vi "GDSAPI_Example_AddDesignPattern.vi"() -> ()   [LabVIEW 2020]
uses:
  GDSAPI_SubVIs/GDSAPI_ClassProviderType.ctl
  ClassProviders/Common/String/GDSString_MethodDescriptionType.ctl
  ClassProviders/Common/CommonVIs/CommonVIs_AttributeType.ctl
  ClassProviders/Common/CommonVIs/CommonVIs_AttributeDataType.ctl
  ClassProviders/Common/String/GDSString_AccessScopeModifierType.ctl
  ClassProviders/Common/String/GDSString_ModifierType.ctl
  ClassProviders/Common/CommonVIs/CommonVIs_PropertyType.ctl
  GDSAPI_CreateClassType.ctl
  GDSAPI_SubVIs/GDSAPI_ClassTemplateType.ctl
  GDSAPI_CreateInterfaceType.ctl
  ClassProviders/Provider_BaseClassInterface/ClassWriter_class/InterfaceMethodsToCreate.ctl
  ClassProviders/Provider_BaseClassInterface/ClassWriter_class/ClassWriter.lvclass
panel:
  out "error out":errorcluster
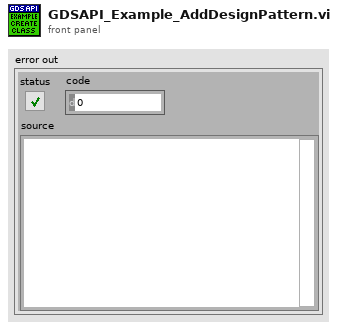
[diagram p1: front panel]
types:
  T1 = typedef "GDSString_MethodDescriptionType.ctl" = cluster{"ReturnType":T2, "MethodName":string, "AccessScope":T4, "Modifiers":T5[], "MethodDocumentation":string, "MethodContent":string, "MethodArguments":T2[], "GetProperty":T6, "SetProperty":T6}
  T2 = typedef "CommonVIs_AttributeType.ctl" = cluster{"Name":string, "DataType":T3, "ArrayDim":i32, "CtrlPath":path, "DataTypeString":string, "AccessScope":T4, "InitialData":variant}
  T3 = typedef "CommonVIs_AttributeDataType.ctl" = enum16{"UINT8", "INT8", "UINT16", "INT16", "UINT32", "INT32", "UINT64", "INT64", "SGL", "DBL", "EXT", "CSG", "CDB", "CXT", "TimeStamp", "STRING", "PATH", "BOOL", "ENUM", "RefNum", "VIRefNum", "LabVIEW Class", "Cluster", "Variant", "TypeDef", "Waveform", "LabVIEW Object", "Other", "void", "Set", "Map"}
  T4 = typedef "GDSString_AccessScopeModifierType.ctl" = enum16{"public", "private", "protected", "internal"}
  T5 = typedef "GDSString_ModifierType.ctl" = enum16{"abstract", "static", "final", "synchronized", "strictfp", "async", "const", "event", "extern", "new", "native ", "override", "partial", "readonly", "sealed", "unsafe", "virtual", "volatile"}
  T6 = typedef "CommonVIs_PropertyType.ctl" = cluster{"Active":bool, "AccessScope":T4, "Code":string}
  T7 = typedef "GDSAPI_ClassProviderType.ctl" = enum16{"LabVIEW Native(By value)", "GOOP-3(By reference)", "GOOP-4(By reference)"}
  T8 = typedef "GDSAPI_CreateInterfaceType.ctl" = cluster{"NewInterfaceFolder":path, "InterfaceName":string, "InterfaceDescription":string, "ParentInterfacesFilePath":path[], "FolderSuffix":string, "MethodsToCreate":T9[]}
  T9 = typedef "ClassWriter.lvclass/InterfaceMethodsToCreate.ctl" = cluster{"Name":string, "Description":string, "MethodsArgumentsIn":T2[], "MethodsArgumentsOut":T2[], "DecendantsMustOverride":bool}
  T10 = typedef "GDSAPI_CreateClassType.ctl" = cluster{"ClassProvider":T7, "NewClassFolder":path, "ParentLvClassFilePath":path, "ClassName":string, "ClassDescription":string, "ClassTemplate":T11, "ParentInterfacesFilePath":path[]}
  T11 = typedef "GDSAPI_ClassTemplateType.ctl" = enum16{"Standard", "Singleton"}
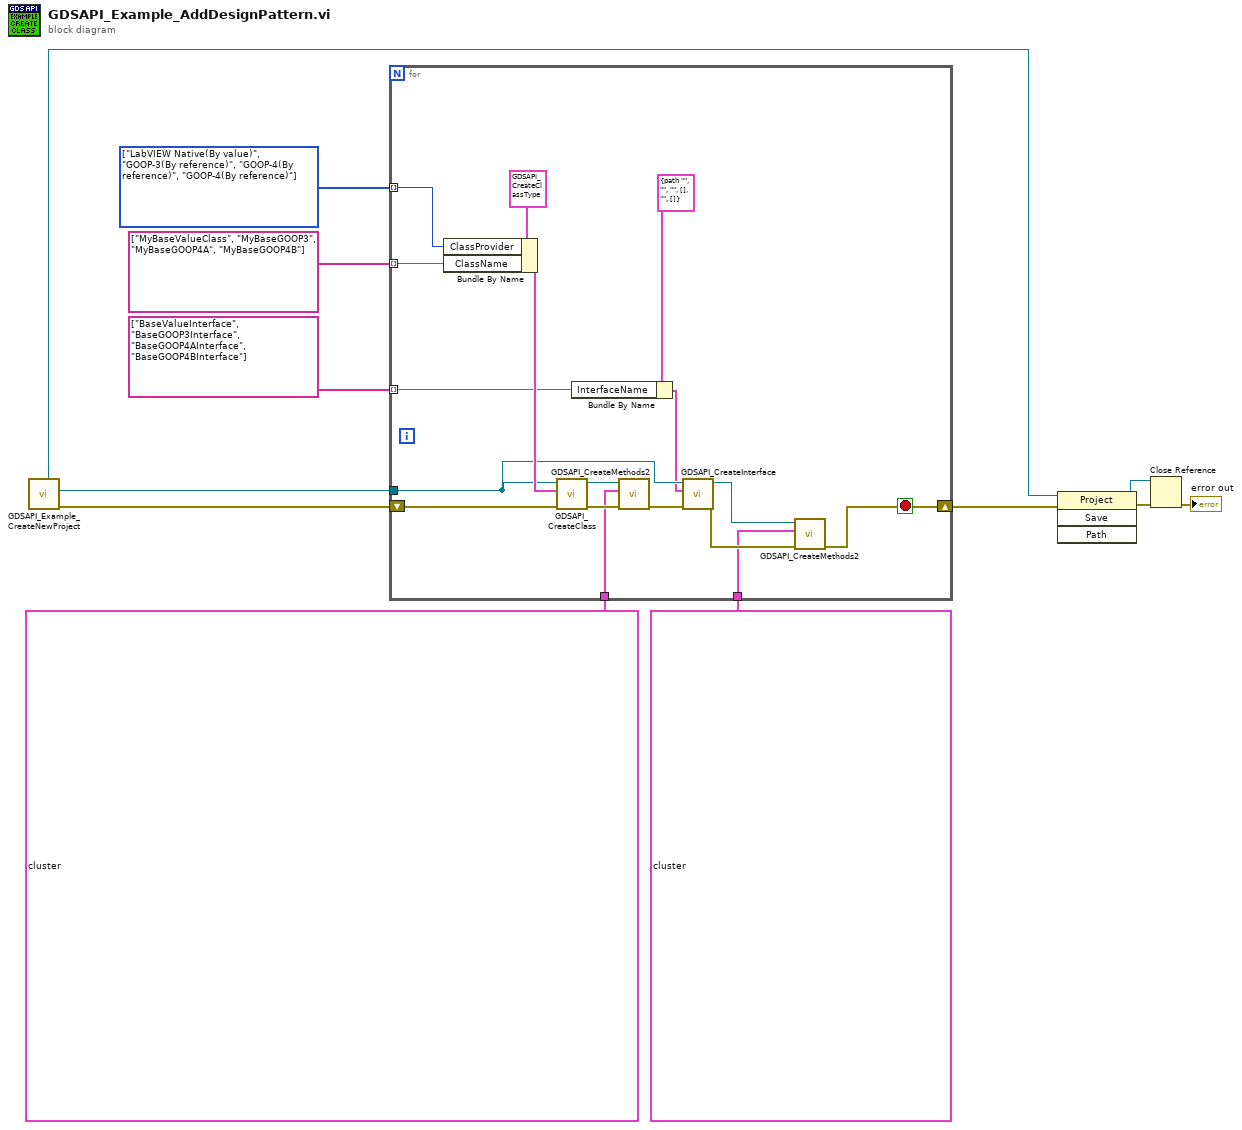
[diagram p0: block diagram]
diagram:
  w7 = T7[] [enum."LabVIEW Native(By value)", enum."GOOP-3(By reference)", enum."GOOP-4(By reference)", enum."GOOP-4(By reference)"] items=["LabVIEW Native(By value)", "GOOP-3(By reference)", "GOOP-4(By reference)"]
  n1 = call "GDSAPI_Example_CreateNewProject.vi"() -> ("error out"=w12:errorcluster, "ProjectItem out"=w11:refnum<vi>, "ProjectRefOut"=w6:refnum<vi>)  [unwired: 8 in, 1 out]
  n2 = for {
    tunnel: w11 -> [w24]
    tunnel: string[] ["MyBaseValueClass", "MyBaseGOOP3", "MyBaseGOOP4A", "MyBaseGOOP4B"] -> [w29] mode=indexing
    tunnel: w7 -> [w28] mode=indexing
    shift-right: [w15] -> w4
    shift-left: w12 -> [w27]
    tunnel: string[] ["BaseValueInterface", "BaseGOOP3Interface", "BaseGOOP4AInterface", "BaseGOOP4BInterface"] -> [w13] mode=indexing
    tunnel: T1[] [{"ReturnType"={"Name"="Message", "DataType"=enum."STRING", "ArrayDim"=0, "CtrlPath"=path "", "DataTypeString"="", "AccessScope"=enum."public", "InitialData"=variant}, "MethodName"="GetMessage", "AccessScope"=enum."public", "Modifiers"=[], "MethodDocumentation"="Doc Doc", "MethodContent"="static void Main()\n{\n    foreach (int number in SomeNumbers())\n    {\n        Console.Write(number.ToString() + \" \");\n    }\n    // Output: 3 5 8\n    Console.ReadKey();\n}", "MethodArguments"=[{"Name"="Get", "DataType"=enum."BOOL", "ArrayDim"=0, "CtrlPath"=path "", "DataTypeString"="", "AccessScope"=enum."public", "InitialData"=variant}], "GetProperty"={"Active"=FALSE, "AccessScope"=enum."public", "Code"=""}, "SetProperty"={"Active"=FALSE, "AccessScope"=enum."public", "Code"=""}}, {"ReturnType"={"Name"="Message", "DataType"=enum."STRING", "ArrayDim"=0, "CtrlPath"=path "", "DataTypeString"="", "AccessScope"=enum."public", "InitialData"=variant}, "MethodName"="GetMessage", "AccessScope"=enum."public", "Modifiers"=[], "MethodDocumentation"="Doc Doc", "MethodContent"="static void Main()\n{\n    foreach (int number in SomeNumbers())\n    {\n        Console.Write(number.ToString() + \" \");\n    }\n    // Output: 3 5 8\n    Console.ReadKey();\n}", "MethodArguments"=[{"Name"="Get", "DataType"=enum."BOOL", "ArrayDim"=0, "CtrlPath"=path "", "DataTypeString"="", "AccessScope"=enum."public", "InitialData"=variant}], "GetProperty"={"Active"=FALSE, "AccessScope"=enum."public", "Code"=""}, "SetProperty"={"Active"=FALSE, "AccessScope"=enum."public", "Code"=""}}] ("Methods") -> [w22]
    tunnel: T1[] [{"ReturnType"={"Name"="Number", "DataType"=enum."DBL", "ArrayDim"=0, "CtrlPath"=path "", "DataTypeString"="", "AccessScope"=enum."public", "InitialData"=variant}, "MethodName"="Do", "AccessScope"=enum."public", "Modifiers"=[], "MethodDocumentation"="My Doc", "MethodContent"=" public int Inventory\n  {\n    get\n    {\n       return _int;\n    }\n    set\n    {\n       // Just to make sure that if there is an increase in inventory then only we are notifying \n          the observers.\n          if (value > _int)\n             Notify();\n          _int = value;\n    }\n  }", "MethodArguments"=[{"Name"="A", "DataType"=enum."UINT8", "ArrayDim"=0, "CtrlPath"=path "", "DataTypeString"="", "AccessScope"=enum."public", "InitialData"=variant}, {"Name"="B", "DataType"=enum."UINT64", "ArrayDim"=1, "CtrlPath"=path "", "DataTypeString"="", "AccessScope"=enum."public", "InitialData"=variant}, {"Name"="C", "DataType"=enum."PATH", "ArrayDim"=0, "CtrlPath"=path "", "DataTypeString"="", "AccessScope"=enum."public", "InitialData"=variant}], "GetProperty"={"Active"=FALSE, "AccessScope"=enum."public", "Code"=""}, "SetProperty"={"Active"=FALSE, "AccessScope"=enum."public", "Code"=""}}] ("Methods") -> [w20]
    stop <- w15 stop-if-true
    n3 = Bundle By Name(cluster=T10 {"ClassProvider"=enum."LabVIEW Native(By value)", "NewClassFolder"=path "", "ParentLvClassFilePath"=path "", "ClassName"="", "ClassDescription"="", "ClassTemplate"=enum."Standard", "ParentInterfacesFilePath"=[]} ("CreateClassType"), "ClassProvider"=w28, "ClassName"=w29) -> (w25:T10)
    n4 = call "GDSAPI_CreateClass.vi"("error in (no error)"=w27, "CreateClassType"=w25, "ProjectItemToCreateClassUnder"=w24) -> ("error out"=w26:errorcluster, "LvClassFileOut"=w18:path)  [unwired: 6 in, 1 out]
    n5 = Bundle By Name(cluster=T8 {"NewInterfaceFolder"=path "", "InterfaceName"="", "InterfaceDescription"="", "ParentInterfacesFilePath"=[], "FolderSuffix"="", "MethodsToCreate"=[]} ("CreateInterfaceType"), "InterfaceName"=w13) -> (w14:T8)
    n6 = call "GDSAPI_CreateMethods2.vi"("error in (no error)"=w26, "Methods"=w22, "ClassPath(*.lvclass)"=w18) -> ("error out"=w23:errorcluster)  [unwired: 7 in, 1 out]
    n7 = call "GDSAPI_CreateInterface.vi"("error in (no error)"=w23, "CreateInterfaceType"=w14, "ProjectItemToCreateClassUnder"=w24) -> ("error out"=w21:errorcluster, "LvClassFileOut"=w19:path)  [unwired: 6 in, 1 out]
    n8 = call "GDSAPI_CreateMethods2.vi"("error in (no error)"=w21, "Methods"=w20, "ClassPath(*.lvclass)"=w19) -> ("error out"=w15:errorcluster)  [unwired: 7 in, 1 out]
  }
  n9 = invoke class="Project" method="Save"(reference=w6, error in=w4) -> (reference out=w9:refnum<vi>, error out=w10:errorcluster)  [unwired: 2 in, 2 out]
  n10 = Close Reference(reference=w9, error in (no error)=w10) -> (error out=→"error out":errorcluster)
